vi "Supervisor_Enter_Fault.vi"(8 "error in (no error)":errorcluster={"status"=FALSE, "code"=0, "source"="\"\""}, 10 "RunContext":string, 11 "FaultRecord":string) -> (0 "error out":errorcluster={"status"=FALSE, "code"=0, "source"="\"\""}, 2 "status ok":bool, 3 "Faulting event and preemption request":string)   [LabVIEW 2026]
doc: "INTENT: Latch global fault and preempt. LOGIC: Latch fault; invalidate all normal owners; cancel all parallel branches; activate protective path first."
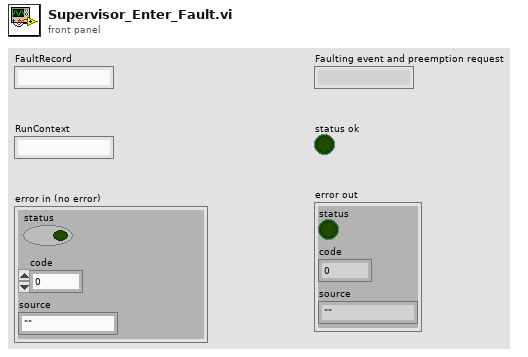
[diagram p1: front panel]
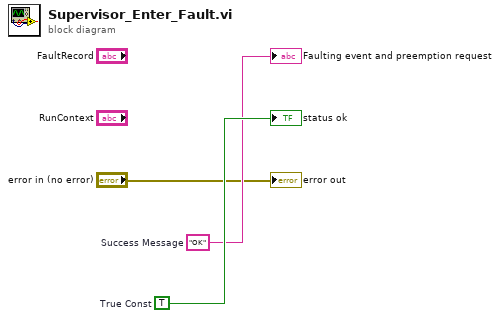
[diagram p0: block diagram]
diagram:
  w3 = TRUE  # True Const
  w2 = "OK"  # Success Message
  "Faulting event and preemption request" <- w2
  "status ok" <- w3
  "error out" <- "error in (no error)"
